vi "GetInterfacesInProject.vi"(8 "error in":errorcluster, 11 "Project/ProjectItem":variant) -> (0 "error out":errorcluster, 2 "InterfaceInfo":T1[](array[typedef]))   [LabVIEW 2020, in "InterfaceLibrary.lvlib"]
uses:
  <resource>/Framework/Providers/Open_GDS/ClassProviders/Common/InterfaceLibrary/InterfaceLibrary.lvlib
  <resource>/Framework/Providers/Open_GDS/ClassProviders/Common/InterfaceLibrary/InterfaceInfo.ctl
  <resource>/Framework/Providers/Open_GDS/ClassProviders/Common/LvClass_class/GDSLvClass_ClassMethodInfo.ctl
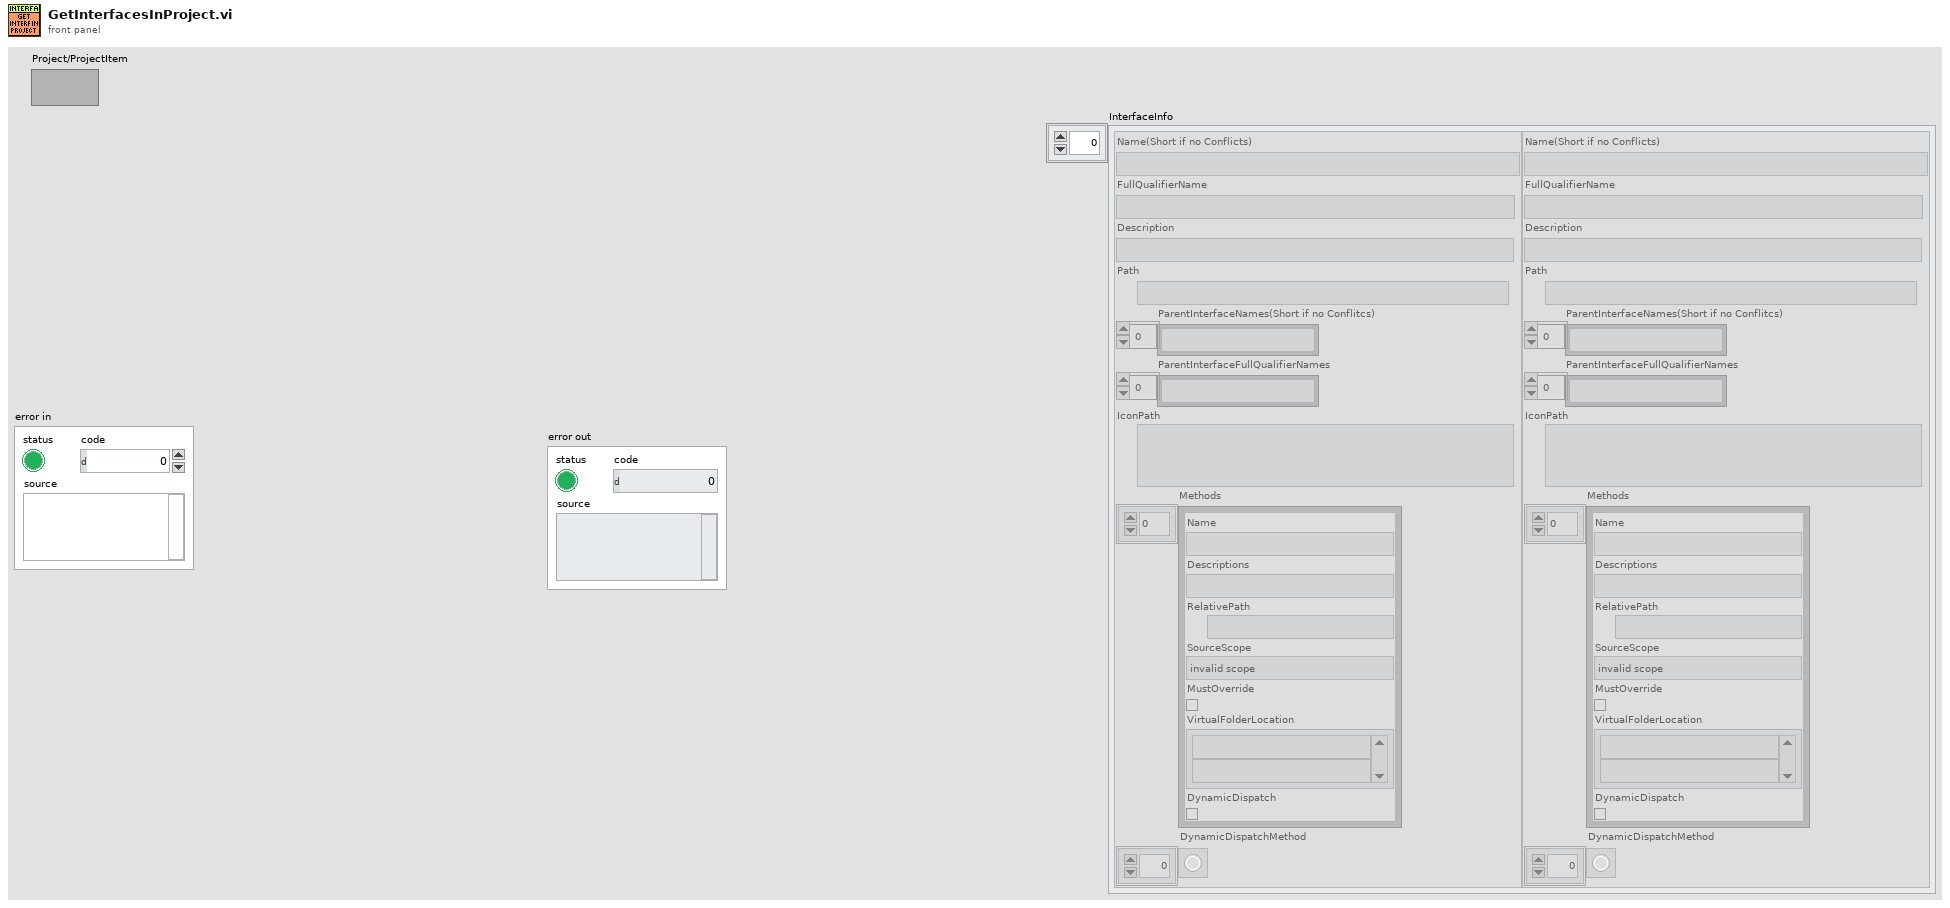
[diagram p1: front panel]
types:
  T1 = typedef "InterfaceLibrary.lvlib/InterfaceInfo.ctl" = cluster{"Name(Short if no Conflicts)":string, "FullQualifierName":string, "Description":string, "Path":path, "ParentInterfaceNames(Short if no Conflitcs)":string[], "ParentInterfaceFullQualifierNames":string[], "IconPath":path, "Methods":T2[], "DynamicDispatchMethod":bool[]}
  T2 = typedef "GDSLvClass_ClassMethodInfo.ctl" = cluster{"Name":string, "Descriptions":string, "RelativePath":path, "SourceScope":enum32{"invalid scope", "public", "private", "protected", "community"}, "MustOverride":bool, "VirtualFolderLocation":string[], "DynamicDispatch":bool}
  T3 = enum32{"invalid scope", "public", "private", "protected", "community"}
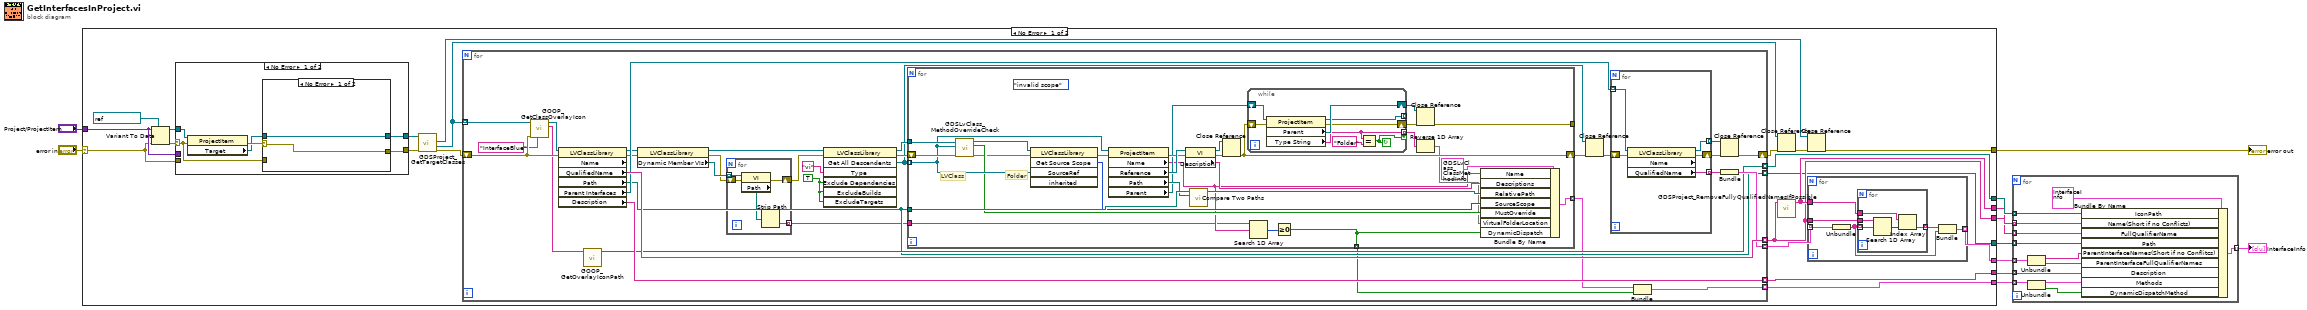
[diagram p0: block diagram]
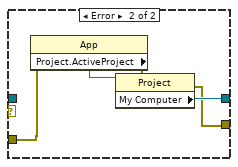
[diagram p2: hidden frame]
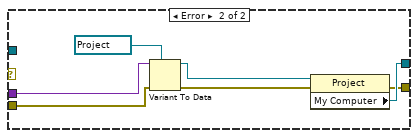
[diagram p3: hidden frame]
diagram:
  n1 = case shown="No Error" "error in" {
    selector: "error in" -> [w28 w143]
    tunnel: "Project/ProjectItem" -> [w29 _]
    tunnel: [w15 w143] -> w9
    tunnel: [w22 _] -> w7
    tunnel: [w21 _] -> w4
    tunnel: [w20 _] -> w6
    tunnel: [w19 _] -> w5
    tunnel: [w18 _] -> w3
    tunnel: [w17 _] -> w8
    tunnel: [w14 _] -> w1
    frame No Error {
      n2 = Variant To Data(error in=w28, type=refnum<vi> refnum ("ProjectItem"), Variant=w29) -> (data=w31:refnum<vi>, error out=w30:errorcluster)
      n3 = case shown="No Error" w30 {
        selector: w30 -> [w123 _]
        tunnel: w31 -> [w128 _]
        tunnel: [w125 w137] -> w27
        tunnel: [w124 w136] -> w26
        tunnel: w29 -> [_ w141]
        tunnel: w28 -> [_ w140]
        frame No Error {
          n4 = property class="ProjectItem"(reference=w128, error in=w123) -> (error out=w127:errorcluster, "Target"=w126:refnum<vi>)  [unwired: 1 out]
          n5 = case shown="No Error" w127 {
            selector: w127 -> [w129 _]
            tunnel: w126 -> [w130 _]
            tunnel: [w130 w134] -> w125
            tunnel: [w129 w131] -> w124
            tunnel: w123 -> [_ w132]
            frame No Error {
            }
            frame Error {
              n6 = property class="App"(error in=w132) -> (error out=w133:errorcluster, "Project.ActiveProject"=w135:refnum<vi>)  [unwired: 1 in, 1 out]
              n7 = property class="Project"(reference=w135, error in=w133) -> (error out=w131:errorcluster, "My Computer"=w134:refnum<vi>)  [unwired: 1 out]
            }
          }
        }
        frame Error {
          n8 = Variant To Data(error in=w140, type=refnum<vi> refnum ("ProjectItem"), Variant=w141) -> (data=w139:refnum<vi>, error out=w138:errorcluster)
          n9 = property class="Project"(reference=w139, error in=w138) -> (error out=w136:errorcluster, "My Computer"=w137:refnum<vi>)  [unwired: 1 out]
        }
      }
      n10 = call <resource>:"GDSProject_GetTargetClasses.vi"("error in (no error)"=w26, "TargetItem in"=w27) -> ("error out"=w25:errorcluster, "LvInterfaces"=w12:refnum<vi>[], "LvClasses"=w13:refnum<vi>[])  [unwired: 4 in, 3 out]
      n11 = for {
        tunnel: w12 -> [w70] mode=indexing
        tunnel: [w75] -> w20 mode=indexing
        shift-right: [w59] -> w24
        shift-left: w25 -> [w68]
        tunnel: [w72] -> w23 mode=indexing
        tunnel: [w54] -> w19 mode=indexing
        tunnel: [w71] -> w18 mode=indexing
        tunnel: [w66] -> w17 mode=indexing
        tunnel: [w53] -> w14 mode=indexing
        w63 = TRUE ("ExcludeDependencies")
        n12 = call <resource>:"GOOP_GetClassOverlayIcon.vi"("DefaultIconName(BlueFull or InterfaceBlue)"="InterfaceBlue" ("DefaultIconName(BlueFull)"), "error in (no error)"=w68, "LVClassLibrary in"=w70) -> ("IconName"=w67:string, "LVClassLibrary out"=w69:refnum<vi>)  [unwired: 6 in, 1 out]
        n13 = property class="LVClassLibrary" props=["Name", "QualifiedName", "Path", "Parent Interfaces", "Description"](reference=w69, error in=w68) -> (reference out=w51:refnum<vi>, error out=w50:errorcluster, "QualifiedName"=w75:string, "Path"=w54:path, "Parent Interfaces"=w74:refnum<vi>[], "Description"=w71:string)  [unwired: 1 out]
        n14 = call <resource>:"GOOP_GetOverlayIconPath.vi"("IconName(NoPngExtension)"=w67) -> ("IconPath"=w66:path)  [unwired: 10 in]
        n15 = property class="LVClassLibrary"(reference=w51, error in=w50) -> (reference out=w49:refnum<vi>, error out=w47:errorcluster, "Dynamic Member VIs"=w48:refnum<vi>[])
        n16 = for {
          tunnel: w48 -> [w80] mode=indexing
          shift-right: [w78] -> w46
          shift-left: w47 -> [w79]
          tunnel: [w76] -> w45 mode=indexing
          n17 = property class="VI"(reference=w80, error in=w79) -> (error out=w78:errorcluster, "Path"=w77:path)  [unwired: 1 out]
          n18 = Strip Path(path=w77) -> (name=w76:string)  [unwired: 1 out]
        }
        n19 = invoke class="LVClassLibrary" method="Get All Descendents"(reference=w49, error in=w46, "Type"="vi", "Exclude Dependencies"=w63, "ExcludeBuilds"=w63, "ExcludeTargets"=w63) -> (reference out=w58:refnum<vi>, error out=w61:errorcluster, "All Descendents"=w55:refnum<vi>[])  [unwired: 1 in, 4 out]
        n20 = for {
          tunnel: w55 -> [w98] mode=indexing
          shift-right: [w95] -> w57
          shift-left: w61 -> [w104]
          tunnel: w58 -> [w105]
          tunnel: w54 -> [w103]
          tunnel: [w93] -> _
          tunnel: [w86] -> w52 mode=indexing
          tunnel: w45 -> [w84]
          tunnel: [w82] -> w44 mode=indexing
          (unwired) T3."invalid scope" ("Source Scope:Get")
          # "Folder"
          # "LVClass"
          n21 = call <resource>:"GDSLvClass_MethodOverrideCheck.vi"("error in (no error)"=w104, "ProjectItem Refnum"=w98, "LVClassLibrary in"=w105) -> ("error out"=w81:errorcluster, "GetMustOverride"=w88:bool, "LVClassLibrary out"=w99:refnum<vi>)  [unwired: 6 in]
          n22 = invoke class="LVClassLibrary" method="Get Source Scope"(reference=w99, error in=w81, "SourceRef"=w98) -> (error out=w97:errorcluster, "GetSourceScope"=w89:T3)  [unwired: 2 in, 3 out]
          n23 = property class="ProjectItem"(reference=w98, error in=w97) -> (error out=w107:errorcluster, "Name"=w85:string, "Reference"=w109:refnum<vi>, "Path"=w102:path, "Parent"=w101:refnum<vi>)  [unwired: 1 out]
          n24 = property class="VI"(reference=w109, error in=w107) -> (reference out=w108:refnum<vi>, error out=w106:errorcluster, "Description"=w91:string)
          n25 = call <vilib>:"Compare Two Paths.vi"("Path 2"=w102, "Path 1"=w103) -> ("Relative Path from 1 to 2"=w90:path)  [unwired: 6 in, 3 out]
          n26 = Close Reference(reference=w108, error in (no error)=w106) -> (error out=w95:errorcluster)
          n27 = while {
            tunnel: [w115] -> w100 mode=indexing if=w113
            shift-right: [w116] -> w96
            shift-left: w101 -> [w117]
            tunnel: [w112] -> _ mode=indexing
            shift-right: [w110] -> w94
            shift-left: w95 -> [w111]
            stop <- w113 continue-if-true
            n28 = property class="ProjectItem"(reference=w117, error in=w111) -> (reference out=w112:refnum<vi>, error out=w110:errorcluster, "Parent"=w116:refnum<vi>, "Type String"=w115:string)
            n29 = Equal?(x=w115, y="Folder") -> (x = y?=w113:bool)
          }
          n30 = Search 1D Array(1D array=w84, element=w85) -> (index of element=w83:i32)  [unwired: 1 in]
          n31 = Greater Or Equal To 0?(x=w83) -> (x >= 0?=w82:bool)
          n32 = Close Reference(reference=w96, error in (no error)=w94) -> (error out=w93:errorcluster)
          n33 = Reverse 1D Array(array=w100) -> (reversed array=w87:string[])
          n34 = Bundle By Name(cluster=T2 {"Name"="", "Descriptions"="", "RelativePath"=path "", "SourceScope"=enum."invalid scope", "MustOverride"=FALSE, "VirtualFolderLocation"=[], "DynamicDispatch"=FALSE} ("MethodSettings"), "Name"=w85, "Descriptions"=w91, "RelativePath"=w90, "SourceScope"=w89, "MustOverride"=w88, "VirtualFolderLocation"=w87, "DynamicDispatch"=w82) -> (w86:T2)
        }
        n35 = Close Reference(reference=w55, error in (no error)=w57) -> (error out=w56:errorcluster)
        n36 = for {
          tunnel: w74 -> [w122] mode=indexing
          tunnel: [w121] -> w73 mode=indexing
          tunnel: [w120] -> w64 mode=indexing
          shift-right: [w118] -> w60
          shift-left: w56 -> [w119]
          n37 = property class="LVClassLibrary" props=["Name", "QualifiedName"](reference=w122, error in=w119) -> (reference out=w120:refnum<vi>, error out=w118:errorcluster, "QualifiedName"=w121:string)  [unwired: 1 out]
        }
        n38 = Bundle(w52, w44) -> (w53:cluster{T2[], bool[]})  [unwired: 1 in]
        n39 = Close Reference(reference=w64, error in (no error)=w60) -> (error out=w59:errorcluster)
        n40 = Bundle(w73) -> (w72:cluster{string[]})  [unwired: 1 in]
      }
      n41 = Close Reference(reference=w12, error in (no error)=w24) -> (error out=w16:errorcluster)
      n42 = call <resource>:"GDSProject_RemoveFullyQualifiedNamesIfPossible.vi"("ItemnamesIn"=w20) -> ("ItemnamesOut"=w22:string[])  [unwired: 10 in]
      n43 = Close Reference(reference=w13, error in (no error)=w16) -> (error out=w15:errorcluster)
      n44 = for {
        tunnel: w23 -> [w38] mode=indexing
        tunnel: w20 -> [w37]
        tunnel: w22 -> [w36]
        tunnel: [w34] -> w21 mode=indexing
        n45 = Unbundle(w38) -> (w33:string[])
        n46 = for {
          tunnel: w33 -> [w43] mode=indexing
          tunnel: w37 -> [w42]
          tunnel: w36 -> [w40]
          tunnel: [w39] -> w35 mode=indexing
          n47 = Search 1D Array(1D array=w42, element=w43) -> (index of element=w41:i32)  [unwired: 1 in]
          n48 = Index Array(array=w40, index=w41) -> (element=w39:string)
        }
        n49 = Bundle(w35, w33) -> (w34:cluster{string[], string[]})  [unwired: 1 in]
      }
    }
    frame Error {
    }
  }
  "error out" <- w9
  n50 = for {
    tunnel: w8 -> [w156] mode=indexing
    tunnel: w7 -> [w155] mode=indexing
    tunnel: w6 -> [w154] mode=indexing
    tunnel: w5 -> [w153] mode=indexing
    tunnel: w4 -> [w152] mode=indexing
    tunnel: w3 -> [w149] mode=indexing
    tunnel: [w147] -> w2 mode=indexing
    tunnel: w1 -> [w146] mode=indexing
    n51 = Unbundle(w146) -> (w145:T2[], w144:bool[])
    n52 = Unbundle(w152) -> (w151:string[], w150:string[])
    n53 = Bundle By Name(cluster=T1 {"Name(Short if no Conflicts)"="", "FullQualifierName"="", "Description"="", "Path"=path "", "ParentInterfaceNames(Short if no Conflitcs)"=[], "ParentInterfaceFullQualifierNames"=[], "IconPath"=path "", "Methods"=[], "DynamicDispatchMethod"=[]} ("InterfaceInfo"), "IconPath"=w156, "Name(Short if no Conflicts)"=w155, "FullQualifierName"=w154, "Path"=w153, "ParentInterfaceNames(Short if no Conflitcs)"=w151, "ParentInterfaceFullQualifierNames"=w150, "Description"=w149, "Methods"=w145, "DynamicDispatchMethod"=w144) -> (w147:T1)
  }
  "InterfaceInfo" <- w2
